vi "Test_Estop_Midrun.vi"(8 "error in":errorcluster, 11 "Sequence Path":path=path "C:/Users/DynaAdmin/PycharmProjects/Universal-sequence-executor-AF/configs/sequences/vtu_actual_sequence.json") -> (0 "error out":errorcluster)   [LabVIEW 2026]
doc: "E-Stop test: Load -> Start -> wait 3s -> Send Emergency Stop (HIGH priority) -> wait 2s -> Normal Stop -> notify. Evidence: results/trace_abort.txt = AB|E-STOP."
uses:
  src/Executor/Sequence Executor.lvclass
  src/Executor Messages/Load Sequence Msg/Load Sequence Msg.lvclass/Load Sequence Msg.ctl
  <vilib>/ActorFramework/Message Enqueuer/Message Enqueuer.lvclass/Message Enqueuer.ctl
  <vilib>/ActorFramework/Message Enqueuer/Enqueue.vi
  src/Executor Messages/Load Sequence Msg/Load Sequence Msg.lvclass
  src/Executor Messages/Start Sequence Msg/Start Sequence Msg.lvclass
  src/Executor Messages/Emergency Stop Msg/Emergency Stop Msg.lvclass
  <vilib>/ActorFramework/Stop Msg/Stop Msg.lvclass
  <vilib>/ActorFramework/Message Priority Queue/Priority Enqueue.vi
  <vilib>/ActorFramework/Actor/Actor.lvclass
panel:
  out "Estop error":errorcluster
  out "Stopped cleanly":bool
  out "Feedback Chart":dbl
  out "Verdict":string
  out "Channel Values":string[][](array[string])
  out "Step Table":string[][](array[string])
  out "Step Index":i32
  out "Status":string
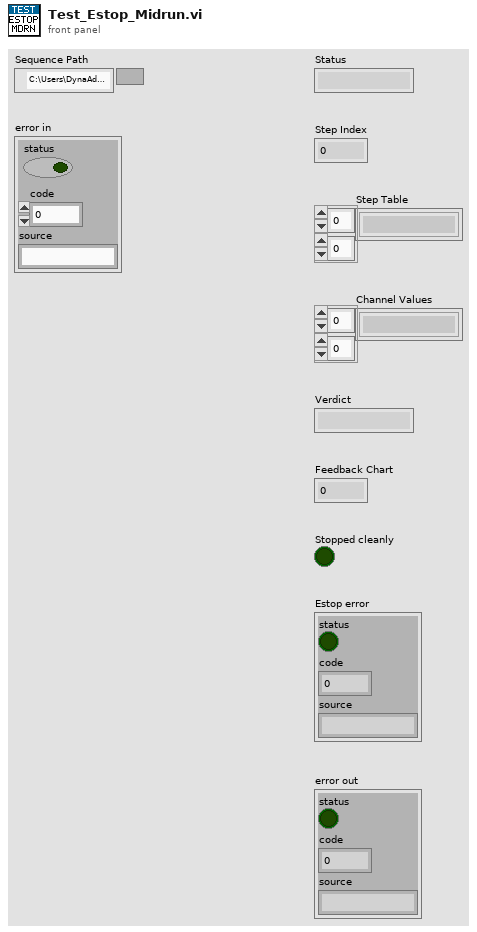
[diagram p1: front panel]
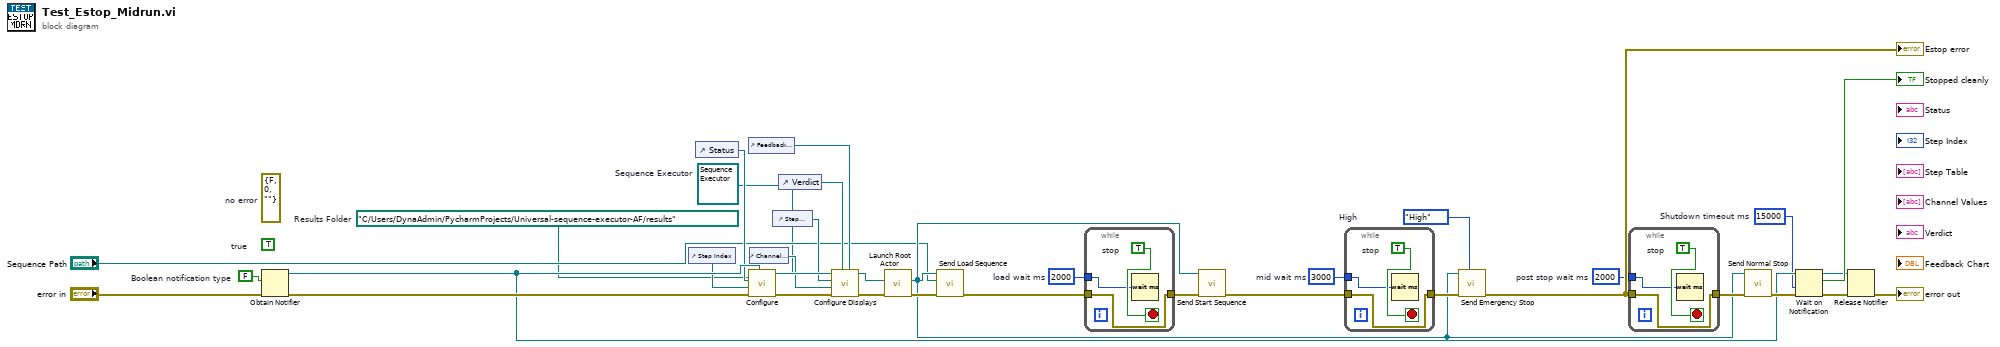
[diagram p0: block diagram]
diagram:
  w8 = enum16{"Low", "Normal", "High"}."High"  # High
  w7 = 2000  # post stop wait ms
  w6 = 3000  # mid wait ms
  w5 = 2000  # load wait ms
  (unwired) TRUE  # true
  w4 = path "C:/Users/DynaAdmin/PycharmProjects/Universal-sequence-executor-AF/results"  # Results Folder
  w3 = 15000  # Shutdown timeout ms
  (unwired) errorcluster {"status"=FALSE, "code"=0, "source"=""}  # no error
  w2 = FALSE  # Boolean notification type
  w1 = refnum<class "Sequence Executor.lvclass"> refnum  # Sequence Executor
  n1 = Obtain Notifier(notification data type=w2, error in (no error)="error in") -> (notifier out=w17:refnum<notifier>, error out=w18:errorcluster)  [unwired: 2 in, 1 out]
  n2 = control-ref of="Step Index"() -> (w12:refnum<vi>)
  n3 = control-ref of="Status"() -> (w11:refnum<vi>)
  n4 = control-ref of="Feedback Chart"() -> (w16:refnum<vi>)
  n5 = call "Configure.vi"("Results Folder"=w4, "Stopped Notification"=w17, "error in"=w18, "Step Index Display"=w12, "Status Display"=w11, "Sequence Executor in"=w1) -> ("error out"=w20:errorcluster, "Sequence Executor out"=w19:refnum<class "Sequence Executor.lvclass">)  [unwired: 4 in]
  n6 = control-ref of="Channel Values"() -> (w14:refnum<vi>)
  n7 = control-ref of="Step Table"() -> (w13:refnum<vi>)
  n8 = control-ref of="Verdict"() -> (w15:refnum<vi>)
  n9 = call "Configure Displays.vi"("Feedback Chart"=w16, "Verdict Display"=w15, "error in"=w20, "Channel Values Display"=w14, "Step Table Display"=w13, "Sequence Executor in"=w19) -> ("error out"=w22:errorcluster, "Sequence Executor out"=w21:refnum<class "Sequence Executor.lvclass">)  [unwired: 4 in]
  n10 = call <vilib>:"Launch Root Actor.vi"("error in (no error)"=w22, "Actor"=w21) -> ("error out"=w24:errorcluster, "Actor's Enqueuer"=w23:refnum<class "Message Enqueuer.lvclass">)  [unwired: 8 in]
  n11 = call "Send Load Sequence.vi"("error in (no error)"=w24, "path"="Sequence Path", "Message Enqueuer"=w23) -> ("error out"=w25:errorcluster)  [unwired: 7 in, 1 out]
  n12 = while {
    tunnel: w5 -> [w37]
    tunnel: w25 -> [w36]
    tunnel: [w36] -> w26
    stop <- w38 stop-if-true
    w38 = TRUE  # stop
    n13 = Wait (ms)(milliseconds to wait=w37) -> ()  [unwired: 1 out]
  }
  n14 = call "Send Start Sequence.vi"("error in (no error)"=w26, "Message Enqueuer"=w23) -> ("error out"=w27:errorcluster)  [unwired: 8 in, 1 out]
  n15 = while {
    tunnel: w6 -> [w40]
    tunnel: w27 -> [w39]
    tunnel: [w39] -> w28
    stop <- w41 stop-if-true
    w41 = TRUE  # stop
    n16 = Wait (ms)(milliseconds to wait=w40) -> ()  [unwired: 1 out]
  }
  n17 = call "Send Emergency Stop.vi"("Message Priority (Normal)"=w8, "error in (no error)"=w28, "Message Enqueuer"=w23) -> ("error out"=w29:errorcluster)  [unwired: 7 in, 1 out]
  "Estop error" <- w29
  n18 = while {
    tunnel: w7 -> [w43]
    tunnel: w29 -> [w42]
    tunnel: [w42] -> w30
    stop <- w44 stop-if-true
    w44 = TRUE  # stop
    n19 = Wait (ms)(milliseconds to wait=w43) -> ()  [unwired: 1 out]
  }
  n20 = call <vilib>:"Send Normal Stop.vi"("error in (no error)"=w30, "Message Enqueuer"=w23) -> ("error out"=w31:errorcluster)  [unwired: 9 in]
  n21 = Wait on Notification(notifier=w17, timeout in ms (-1)=w3, error in (no error)=w31) -> (notifier out=w32:refnum<notifier>, notification=→"Stopped cleanly":bool, error out=w34:errorcluster)  [unwired: 1 in, 1 out]
  n22 = Release Notifier(notifier=w32, error in (no error)=w34) -> (error out=→"error out":errorcluster)  [unwired: 1 in, 2 out]
